vi "Day 3.vi"() -> ()   [LabVIEW 2021]
uses:
  <vilib>/Utility/file.llb/Read Delimited Spreadsheet (string).vi
panel:
  out "x*y":i32
  out "subarray":string[](array[string])
  in  "Input File":enum32{"example input", "input"}(radio)
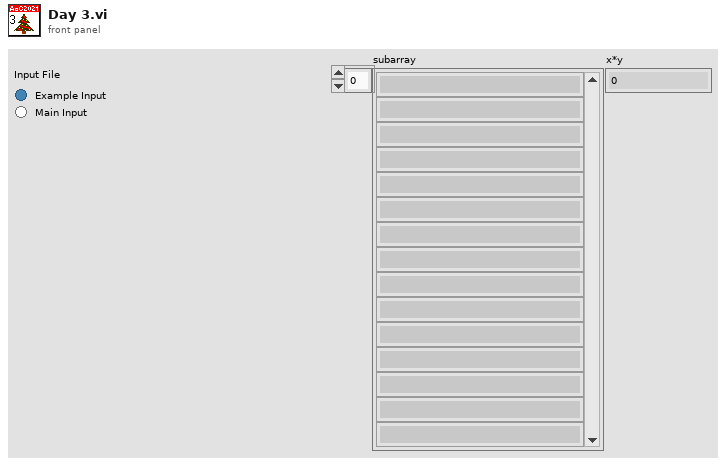
[diagram p1: front panel]
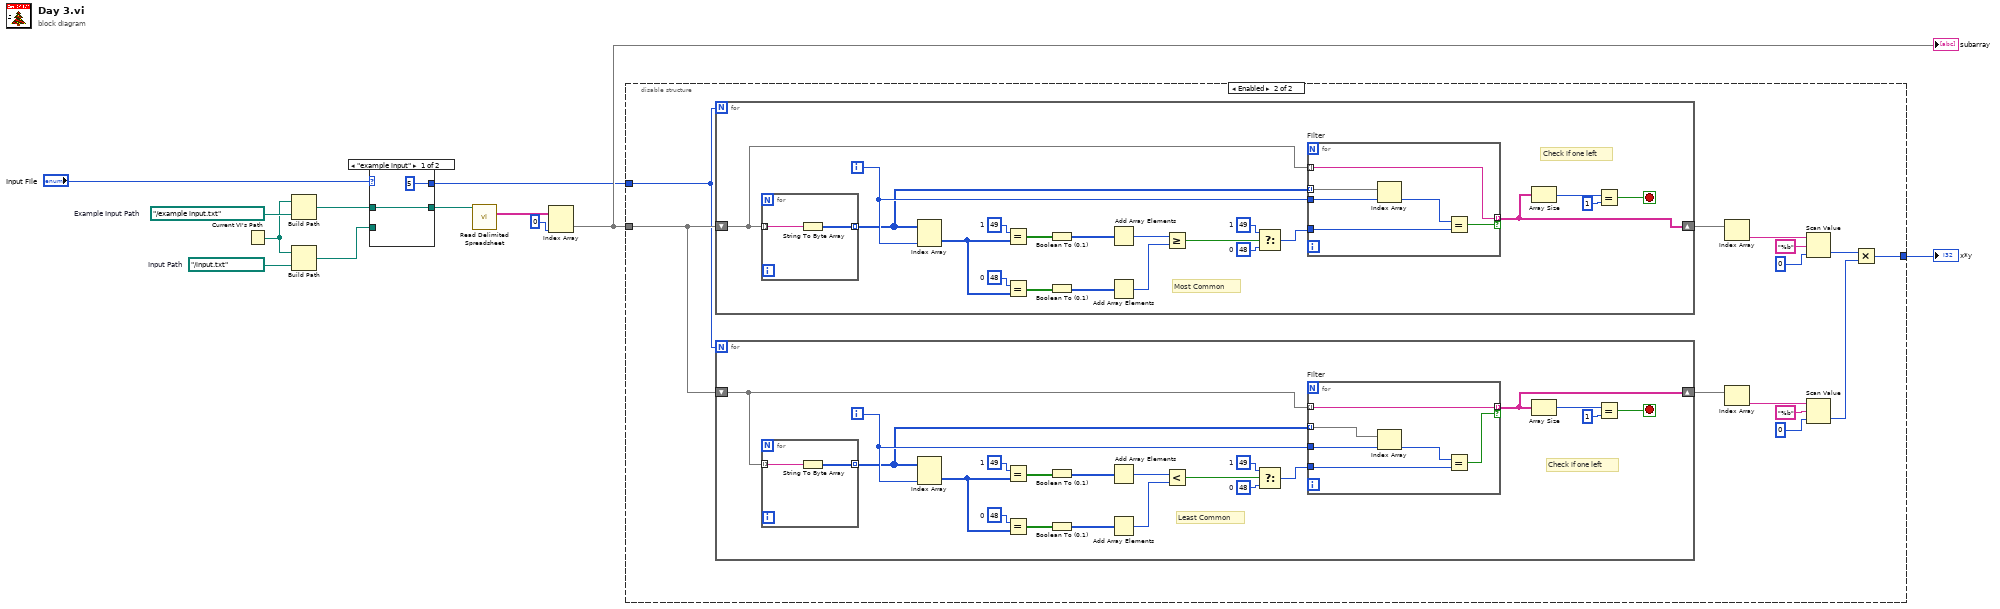
[diagram p0: block diagram]
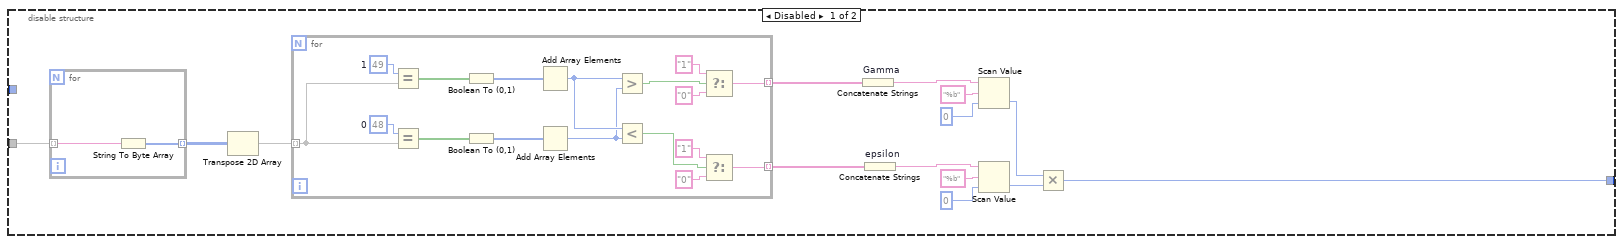
[diagram p2: hidden frame]
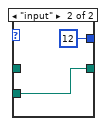
[diagram p3: hidden frame]
diagram:
  w11 = path "../example input.txt"  # Example Input Path
  w12 = path "../input.txt"  # Input Path
  n1 = Current VI's Path() -> (path=w6:path)
  n2 = Build Path(base path=w6, name or relative path=w11) -> (appended path=w8:path)
  n3 = Build Path(base path=w6, name or relative path=w12) -> (appended path=w9:path)
  n4 = case shown="\"example input\"" "Input File" {
    tunnel: w9 -> [_ w16]
    tunnel: w8 -> [w14 _]
    tunnel: [w14 w16] -> w7
    tunnel: [5 12] -> w1
    frame "example input" {
    }
    frame "input" {
    }
  }
  n5 = call-poly <vilib>:"Read Delimited Spreadsheet.vi"("file path (dialog if empty)"=w7) -> ("all rows"=w5:string[][])  [unwired: 9 in, 5 out]
  n6 = Index Array(array=w5, index (col)=0 ("disabled index (col)")) -> (element=w3:string[])  [unwired: 1 in]
  "subarray" <- w3
  n7 = disable-structure shown="Enabled" {
    disable-tunnel: w3 -> [w30 w61]
    disable-tunnel: [w17 w62] -> w2
    disable-tunnel: w1 -> [_ w50]
    frame Disabled {
      n8 = for {
        tunnel: w30 -> [w49] mode=indexing
        tunnel: [w48] -> w29 mode=indexing
        n9 = String To Byte Array(string=w49) -> (unsigned byte array=w48:u8[])
      }
      n10 = Transpose 2D Array(2D array=w29) -> (transposed array=w28:u8[][])
      n11 = for {
        tunnel: w28 -> [w45] mode=indexing
        tunnel: [w32] -> w26 mode=indexing
        tunnel: [w31] -> w27 mode=indexing
        w46 = 48  # 0
        w47 = 49  # 1
        n12 = Equal?(x=w47, y=w45) -> (x = y?=w44:bool[])
        n13 = Equal?(x=w46, y=w45) -> (x = y?=w43:bool[])
        n14 = Boolean To (0,1)(Boolean=w44) -> (0, 1=w42:i16[])
        n15 = Boolean To (0,1)(Boolean=w43) -> (0, 1=w41:i16[])
        n16 = Add Array Elements(numeric array=w42) -> (sum=w37:i16)
        n17 = Add Array Elements(numeric array=w41) -> (sum=w36:i16)
        n18 = Greater?(x=w37, y=w36) -> (0:w40:bool)
        n19 = Less?(x=w37, y=w36) -> (x < y?=w33:bool)
        n20 = Select(t="1", s=w40, f="0") -> (s? t:f=w31:string)
        n21 = Select(t="1", s=w33, f="0") -> (s? t:f=w32:string)
      }
      n22 = Concatenate Strings "Gamma"(w27) -> (w25:string)
      n23 = Concatenate Strings "epsilon"(w26) -> (w20:string)
      n24 = Scan Value(string=w25, format string="%b", default (0 dbl)=0) -> (value=w19:i32)  [unwired: 1 out]
      n25 = Scan Value(string=w20, format string="%b", default (0 dbl)=0) -> (value=w18:i32)  [unwired: 1 out]
      n26 = Multiply(x=w19, y=w18) -> (x*y=w17:i32)
    }
    frame Enabled {
      n27 = for {
        N: w50 -> [_]
        shift-right: [w66] -> w55
        shift-left: w61 -> [w64]
        i -> [w65]
        stop <- w67 stop-if-true
        w71 = 48  # 0
        w72 = 49  # 1
        w80 = 48  # 0
        w81 = 49  # 1
        # "Most Common"
        # "Check if one left"
        n28 = for {
          tunnel: w64 -> [w84] mode=indexing
          tunnel: [w83] -> w63 mode=indexing
          n29 = String To Byte Array(string=w84) -> (unsigned byte array=w83:u8[])
        }
        n30 = Index Array(array=w63, index (col)=w65) -> (element=w82:u8[])  [unwired: 1 in]
        n31 = Equal?(x=w81, y=w82) -> (x = y?=w79:bool[])
        n32 = Equal?(x=w80, y=w82) -> (x = y?=w78:bool[])
        n33 = Boolean To (0,1)(Boolean=w79) -> (0, 1=w77:i16[])
        n34 = Boolean To (0,1)(Boolean=w78) -> (0, 1=w76:i16[])
        n35 = Add Array Elements(numeric array=w77) -> (sum=w75:i16)
        n36 = Add Array Elements(numeric array=w76) -> (sum=w74:i16)
        n37 = Greater Or Equal?(x=w75, y=w74) -> (x >= y?=w73:bool)
        n38 = Select(t=w72, s=w73, f=w71) -> (s? t:f=w70:i32)
        n39 = for "Filter" {
          tunnel: w63 -> [w90] mode=indexing
          tunnel: w70 -> [w89]
          tunnel: w64 -> [w87] mode=indexing
          tunnel: [w87] -> w66 mode=indexing if=w88
          tunnel: w65 -> [w85]
          n40 = Index Array(array=w90, index=w85) -> (element=w86:u8)
          n41 = Equal?(x=w86, y=w89) -> (x = y?=w88:bool)
        }
        n42 = Array Size(array=w66) -> (size(s)=w69:i32)
        n43 = Equal?(x=w69, y=1) -> (x = y?=w67:bool)
      }
      n44 = for {
        N: w50 -> [_]
        shift-right: [w94] -> w60
        shift-left: w61 -> [w92]
        i -> [w93]
        stop <- w95 stop-if-true
        w99 = 49  # 1
        w100 = 48  # 0
        w108 = 48  # 0
        w109 = 49  # 1
        # "Least Common"
        # "Check if one left"
        n45 = for {
          tunnel: w92 -> [w112] mode=indexing
          tunnel: [w111] -> w91 mode=indexing
          n46 = String To Byte Array(string=w112) -> (unsigned byte array=w111:u8[])
        }
        n47 = Index Array(array=w91, index (col)=w93) -> (element=w110:u8[])  [unwired: 1 in]
        n48 = Equal?(x=w109, y=w110) -> (x = y?=w107:bool[])
        n49 = Equal?(x=w108, y=w110) -> (x = y?=w106:bool[])
        n50 = Boolean To (0,1)(Boolean=w107) -> (0, 1=w105:i16[])
        n51 = Boolean To (0,1)(Boolean=w106) -> (0, 1=w104:i16[])
        n52 = Add Array Elements(numeric array=w105) -> (sum=w103:i16)
        n53 = Add Array Elements(numeric array=w104) -> (sum=w102:i16)
        n54 = Less?(x=w103, y=w102) -> (x < y?=w101:bool)
        n55 = Select(t=w99, s=w101, f=w100) -> (s? t:f=w98:i32)
        n56 = for "Filter" {
          tunnel: w91 -> [w118] mode=indexing
          tunnel: w98 -> [w117]
          tunnel: w92 -> [w115] mode=indexing
          tunnel: [w115] -> w94 mode=indexing if=w116
          tunnel: w93 -> [w113]
          n57 = Index Array(array=w118, index=w113) -> (element=w114:u8)
          n58 = Equal?(x=w114, y=w117) -> (x = y?=w116:bool)
        }
        n59 = Array Size(array=w94) -> (size(s)=w97:i32)
        n60 = Equal?(x=w97, y=1) -> (x = y?=w95:bool)
      }
      n61 = Index Array(array=w55) -> (element=w52:string)  [unwired: 1 in]
      n62 = Index Array(array=w60) -> (element=w59:string)  [unwired: 1 in]
      n63 = Scan Value(string=w52, format string="%b", default (0 dbl)=0) -> (value=w51:i32)  [unwired: 1 out]
      n64 = Scan Value(string=w59, format string="%b", default (0 dbl)=0) -> (value=w56:i32)  [unwired: 1 out]
      n65 = Multiply(x=w51, y=w56) -> (x*y=w62:i32)
    }
  }
  "x*y" <- w2
